vi "RemoteVI Swallow Button Up.vi"(0 "posts":cluster{"msg":u32, "wParam":u64, "lParam":i64}[](array[cluster])) -> (4 "posts out":cluster{"msg":u32, "wParam":u64, "lParam":i64}[](array[cluster]))   [LabVIEW 2020, in "RemoteVI.lvlib"]
doc: "Drops the button-up of a click that RemoteVI Menu Click.vi turned into keys (docs\\architecture.md, Popups): the button-down chose a menu item with VK_RETURN, the menu closed, and the up would otherwise reach the panel as a stray WM_xBUTTONUP at whatever control lies under the menu. When posts starts with a button-up (WM_LBUTTONUP 514, WM_RBUTTONUP 517, WM_MBUTTONUP 520) and the menu pointer state (RemoteVI Menu Pointer.vi) has swallow up set, posts out is empty. Any button-up or button-down clears swallow up, so at most the one next up is dropped. Otherwise posts passes through."
uses:
  RemoteVI.lvlib
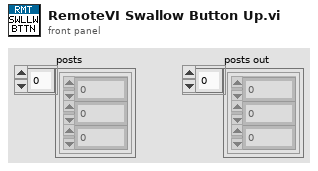
[diagram p1: front panel]
types:
  T1 = cluster{"active":bool, "x":i32, "y":i32, "moved":u32, "navigated":bool, "menu":u64, "top":i32, "hit":bool, "row since":u32, "dwelled":bool, "plain":u64, "swallow up":bool}
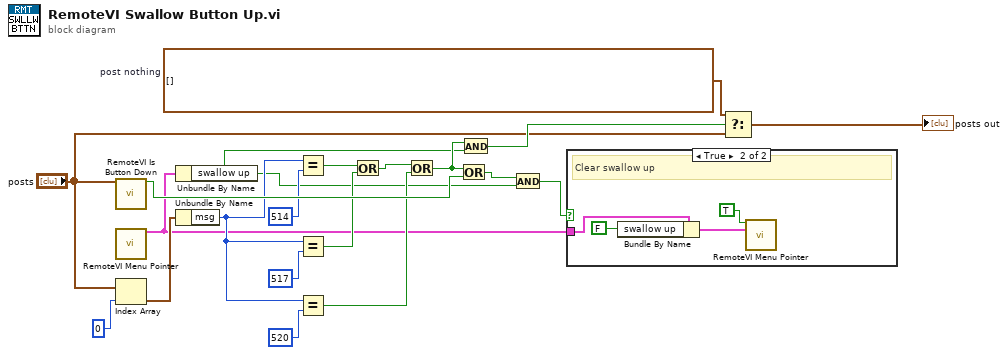
[diagram p0: block diagram]
diagram:
  w19 = cluster{"msg":u32, "wParam":u64, "lParam":i64}[] []  # post nothing
  n1 = call "RemoteVI Is Button Down.vi"("posts"="posts") -> ("button down?"=w15:bool)  [unwired: 14 in]
  n2 = call "RemoteVI Menu Pointer.vi"() -> ("state"=w2:T1)  [unwired: 15 in]
  n3 = Index Array(array="posts", index=0) -> (element=w5:cluster{"msg":u32, "wParam":u64, "lParam":i64})
  n4 = Unbundle By Name(w2) -> ("swallow up"=w3:bool)
  n5 = Unbundle By Name(w5) -> ("msg"=w6:u32)
  n6 = Equal?(x=w6, y=u32 514) -> (x = y?=w10:bool)
  n7 = Equal?(x=w6, y=u32 517) -> (x = y?=w11:bool)
  n8 = Equal?(x=w6, y=u32 520) -> (x = y?=w12:bool)
  n9 = Or(x=w10, y=w11) -> (x .or. y?=w13:bool)
  n10 = Or(x=w13, y=w12) -> (x .or. y?=w14:bool)
  n11 = Or(x=w14, y=w15) -> (x .or. y?=w17:bool)
  n12 = And(x=w14, y=w3) -> (x .and. y?=w16:bool)
  n13 = And(x=w17, y=w3) -> (x .and. y?=w18:bool)
  n14 = case shown="True" w18 {
    tunnel: w2 -> [_ w21]
    frame False {
    }
    frame True {
      # "Clear swallow up"
      n15 = Bundle By Name(cluster=w21, "swallow up"=FALSE) -> (w24:T1)
      n16 = call "RemoteVI Menu Pointer.vi"("write?"=TRUE, "state in"=w24) -> ()  [unwired: 13 in, 1 out]
    }
  }
  n17 = Select(t=w19, s=w16, f="posts") -> (s? t:f=→"posts out":cluster{"msg":u32, "wParam":u64, "lParam":i64}[])
